vi "RemoteVI Track Windows.vi"(0 "look?":bool, 1 "now":u32, 2 "last list":u32, 5 "panel hWnd":u64, 7 "state":T1, 9 "previous windows":T2(array[cluster]), 11 "other shares":u64[](array[numeric])) -> (3 "last list out":u32, 4 "windows":T2(array[cluster]), 6 "message":string, 8 "modal?":bool, 10 "state out":T1)   [LabVIEW 2020, in "RemoteVI.lvlib"]
doc: "The windows part of one server loop iteration (docs\\protocol.md section 7). When look? is TRUE (a client is connected, the geometry is due or a popup was open) or a modal window was listed last time, and at least 200 ms after the last listing (last list - listing walks every top-level window of the desktop, about 12 ms in the IDE, measured; every iteration would make each iteration a frame iteration, and the OVERLAY, which goes out in the iterations between frames, would starve), the application's other windows are listed (RemoteVI List Windows.vi - Win32 only, so it runs while a dialog holds LabVIEW's UI thread); otherwise the previous list is kept. Candidates that just appeared and are not listed are passed to RemoteVI Running Panels.vi (VI Server, so only while no modal window is listed); those that are open front panels of running VIs - the application's own non-modal windows, such as a subVI panel opened with FP.Open - are added to the listed set of state out and so listed from the next listing on, while IDE windows stay unlisted. message is the text message windows [...] of the list (RemoteVI Windows Message.vi), modal? is TRUE while a listed window is modal - LabVIEW's UI thread then runs a dialog's modal loop and every VI Server UI call would block until it closes (measured on LabVIEW 2025 with a Two Button Dialog), so the server loop makes none."
uses:
  RemoteVI.lvlib
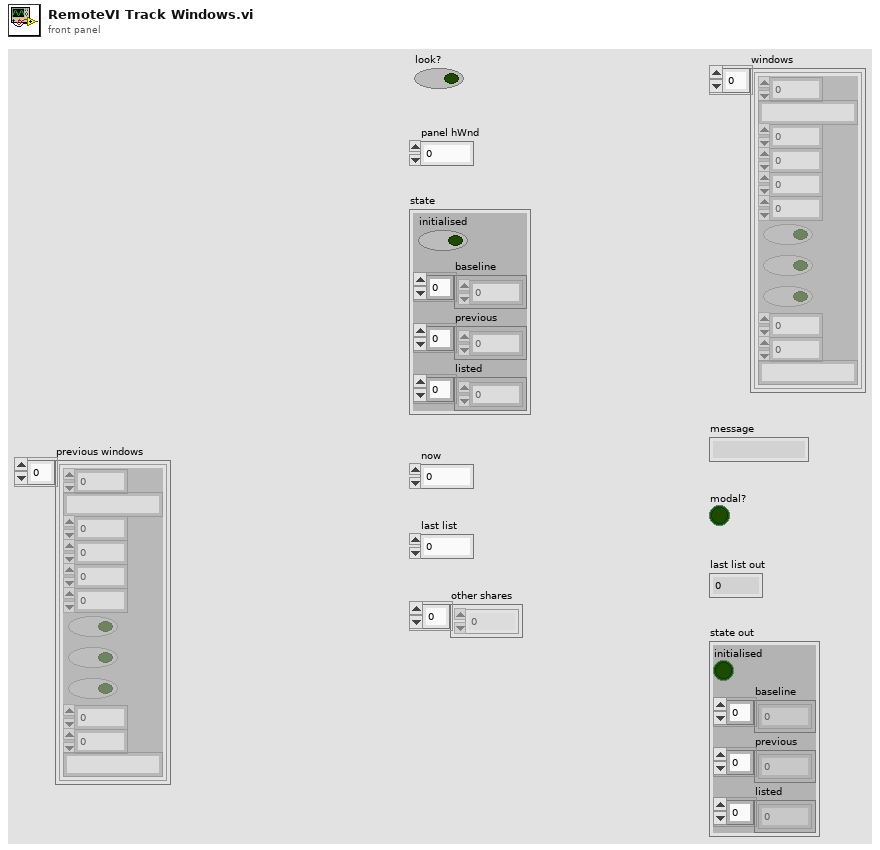
[diagram p1: front panel]
types:
  T1 = cluster{"initialised":bool, "baseline":u64[], "previous":u64[], "listed":u64[]}
  T2 = cluster{"id":u64, "title":string, "x":i32, "y":i32, "w":i32, "h":i32, "modal":bool, "active":bool, "closable":bool, "sx":i32, "sy":i32, "class":string}[]
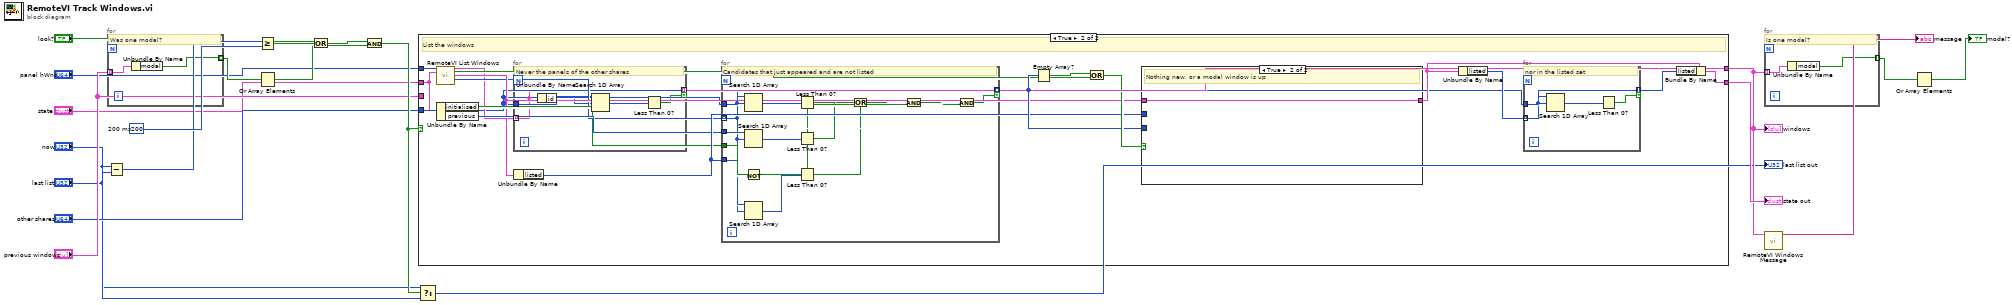
[diagram p0: block diagram]
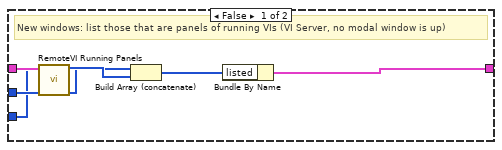
[diagram p3: hidden frame]
diagram:
  w12 = u32 200  # 200 ms
  n1 = for {
    tunnel: "previous windows" -> [w21] mode=indexing
    tunnel: [w22] -> w8 mode=indexing
    # "Was one modal?"
    n2 = Unbundle By Name(w21) -> ("modal"=w22:bool)
  }
  n3 = Subtract(x="now", y="last list") -> (x-y=w11:u32)
  n4 = Greater Or Equal?(x=w11, y=w12) -> (x >= y?=w13:bool)
  n5 = Or Array Elements(Boolean array=w8) -> (logical OR=w9:bool)
  n6 = Or(x="look?", y=w9) -> (x .or. y?=w10:bool)
  n7 = And(x=w10, y=w13) -> (x .and. y?=w14:bool)
  n8 = case shown="True" w14 {
    tunnel: "panel hWnd" -> [_ w25]
    tunnel: "state" -> [w23 w26]
    tunnel: "previous windows" -> [w24 _]
    tunnel: "other shares" -> [_ w27]
    tunnel: [w24 w39] -> w16
    tunnel: [w23 w42] -> w17
    frame False {
      # "Keep the previous list"
    }
    frame True {
      # "List the windows"
      n9 = call "RemoteVI List Windows.vi"("panel hWnd"=w25, "state"=w26) -> ("windows"=w28:T2, "modal?"=w29:bool, "state out"=w31:T1, "candidates"=w30:u64[])  [unwired: 9 in, 1 out]
      n10 = Unbundle By Name(w26) -> ("initialised"=w32:bool, "previous"=w33:u64[])
      n11 = for {
        tunnel: w27 -> [w48]
        tunnel: w28 -> [w47] mode=indexing
        tunnel: [w47] -> w39 mode=indexing if=w51
        # "Never the panels of the other shares"
        n12 = Unbundle By Name(w47) -> ("id"=w49:u64)
        n13 = Search 1D Array(1D array=w48, element=w49) -> (index of element=w50:i32)  [unwired: 1 in]
        n14 = Less Than 0?(x=w50) -> (x < 0?=w51:bool)
      }
      n15 = Unbundle By Name(w31) -> ("listed"=w34:u64[])
      n16 = for {
        tunnel: w27 -> [w63]
        tunnel: w30 -> [w59] mode=indexing
        tunnel: w33 -> [w60]
        tunnel: w32 -> [w62]
        tunnel: w34 -> [w61]
        tunnel: [w59] -> w35 mode=indexing if=w73
        # "Candidates that just appeared and are not listed"
        n17 = Search 1D Array(1D array=w63, element=w59) -> (index of element=w64:i32)  [unwired: 1 in]
        n18 = Search 1D Array(1D array=w60, element=w59) -> (index of element=w66:i32)  [unwired: 1 in]
        n19 = Not(x=w62) -> (.not. x?=w68:bool)
        n20 = Search 1D Array(1D array=w61, element=w59) -> (index of element=w70:i32)  [unwired: 1 in]
        n21 = Less Than 0?(x=w64) -> (x < 0?=w65:bool)
        n22 = Less Than 0?(x=w66) -> (x < 0?=w67:bool)
        n23 = Less Than 0?(x=w70) -> (x < 0?=w71:bool)
        n24 = Or(x=w67, y=w68) -> (x .or. y?=w69:bool)
        n25 = And(x=w69, y=w71) -> (x .and. y?=w72:bool)
        n26 = And(x=w72, y=w65) -> (x .and. y?=w73:bool)
      }
      n27 = Empty Array?(array=w35) -> (empty?=w36:bool)
      n28 = Or(x=w36, y=w29) -> (x .or. y?=w37:bool)
      n29 = case shown="True" w37 {
        tunnel: w31 -> [w53 w58]
        tunnel: w34 -> [w54 _]
        tunnel: w35 -> [w52 _]
        tunnel: [w57 w58] -> w38
        frame False {
          # "New windows: list those that are panels of running VIs (VI Server, no modal window is up)"
          n30 = call "RemoteVI Running Panels.vi"("hWnds"=w52) -> ("running panels"=w55:u64[])  [unwired: 13 in, 1 out]
          n31 = Build Array (concatenate)(w54, w55) -> (w56:u64[])
          n32 = Bundle By Name(cluster=w53, "listed"=w56) -> (w57:T1)
        }
        frame True {
          # "Nothing new, or a modal window is up"
        }
      }
      n33 = Unbundle By Name(w38) -> ("listed"=w40:u64[])
      n34 = for {
        tunnel: w27 -> [w44]
        tunnel: w40 -> [w43] mode=indexing
        tunnel: [w43] -> w41 mode=indexing if=w46
        # "nor in the listed set"
        n35 = Search 1D Array(1D array=w44, element=w43) -> (index of element=w45:i32)  [unwired: 1 in]
        n36 = Less Than 0?(x=w45) -> (x < 0?=w46:bool)
      }
      n37 = Bundle By Name(cluster=w38, "listed"=w41) -> (w42:T1)
    }
  }
  "windows" <- w16
  "state out" <- w17
  n38 = Select(t="now", s=w14, f="last list") -> (s? t:f=→"last list out":u32)
  n39 = for {
    tunnel: w16 -> [w74] mode=indexing
    tunnel: [w75] -> w18 mode=indexing
    # "Is one modal?"
    n40 = Unbundle By Name(w74) -> ("modal"=w75:bool)
  }
  n41 = call "RemoteVI Windows Message.vi"("windows"=w16) -> ("message"=→"message":string)  [unwired: 14 in]
  n42 = Or Array Elements(Boolean array=w18) -> (logical OR=→"modal?":bool)
